vi "Test_simu_banc.vi"() -> ()   [LabVIEW 2026]
panel:
  out "R%":dbl
  out "Nb KO":i32
  out "Nb OK":i32
  in  "stop":bool
  out "Boolean":bool
  out "Waveform Chart":dbl(graph)
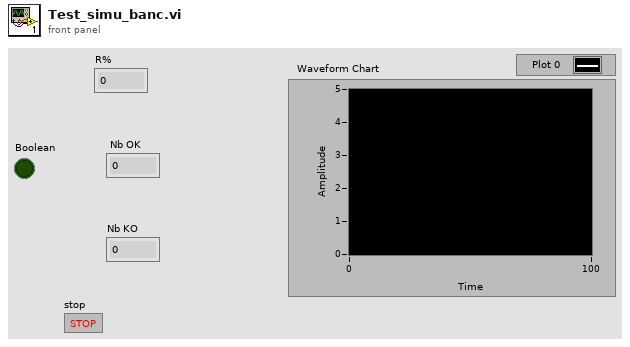
[diagram p1: front panel]
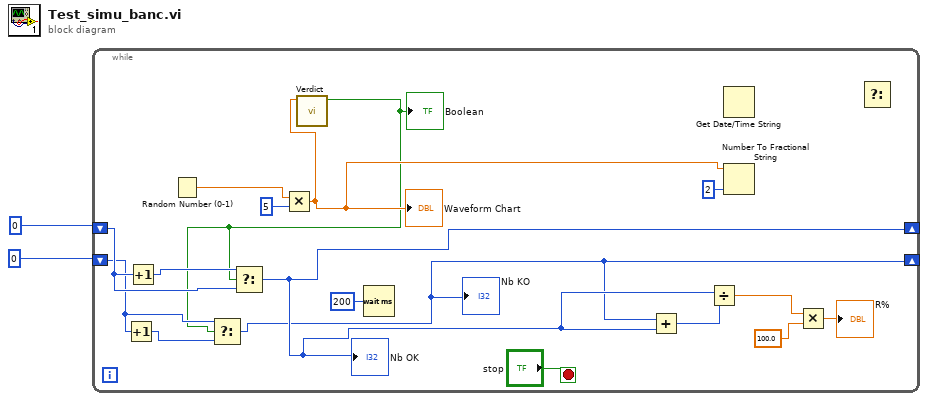
[diagram p0: block diagram]
diagram:
  n1 = while {
    shift-right: [w4] -> _
    shift-left: 0 -> [w14]
    shift-right: [w3] -> _
    shift-left: 0 -> [w8]
    stop <- "stop" stop-if-true
    n2 = Increment(x=w8) -> (x+1=w9:i32)
    n3 = Increment(x=w14) -> (x+1=w15:i32)
    n4 = Random Number (0-1)() -> (number: 0 to 1=w17:dbl)
    n5 = Multiply(x=w17, y=u64 5) -> (x*y=w7:dbl)
    "Waveform Chart" <- w7
    n6 = call "Verdict.vi"("Tension"=w7) -> ("OK"=w5:bool)  [unwired: 10 in]
    "Boolean" <- w5
    n7 = Select(t=w8, s=w5, f=w9) -> (s? t:f=w3:i32)
    "Nb KO" <- w3
    n8 = Select(t=w15, s=w5, f=w14) -> (s? t:f=w4:i32)
    "Nb OK" <- w4
    n9 = Wait (ms)(milliseconds to wait=u32 200) -> ()  [unwired: 1 out]
    n10 = Add(x=w3, y=w4) -> (x+y=w13:i32)
    n11 = Divide(x=w4, y=w13) -> (x/y=w12:dbl)
    n12 = Get Date/Time String() -> ()  [unwired: 3 in, 2 out]
    n13 = Number To Fractional String(number=w7, precision (6)=i16 2) -> ()  [unwired: 2 in, 1 out]
    n14 = Multiply(x=w12, y=100.0) -> (x*y=→"R%":dbl)
    n15 = Select() -> ()  [unwired: 3 in, 1 out]
  }
